vi "Test Streaming.vi"() -> ()   [LabVIEW 2021]
uses:
  <vilib>/CIF Foundation/CIF CAN RW Core/typedef/CAN Port Configuration.ctl
  <vilib>/CIF Foundation/CIF CAN RW Core/typedef/CAN Mode.ctl
  <vilib>/CIF Foundation/CIF CAN RW Core/typedef/FD Config.ctl
  <vilib>/xnet/xnet.llb/XNET Frame CAN.ctl
  <vilib>/xnet/xnet.llb/XNET Frame Type CAN.ctl
  <vilib>/CIF Foundation/CIF CAN RW Core/typedef/Statistics.ctl
  XNET CAN RW.lvclass
  C:/Program Files/National Instruments/LabVIEW 2021/vi.lib/CIF Foundation/CIF CAN RW Core/CAN_RW_CORE.lvclass
  <vilib>/CIF Foundation/CIF CAN RW Core/CAN_RW_CORE.lvclass/CAN_RW_CORE.ctl
  <vilib>/CIF Foundation/CIF CAN RW Core/Accessors/Write One Shot TX.vi
  <vilib>/CIF Foundation/CIF CAN RW Core/CAN_RW_CORE.lvclass
  D:/dev/Packages/CAN_RW_XNET/src/XNET CAN RW.lvclass
  <vilib>/CIF Foundation/CIF CAN RW Core/typedef/Communication State.ctl
  <vilib>/CIF Foundation/CIF CAN RW Core/typedef/Last Error.ctl
  <vilib>/CIF Foundation/CIF CAN RW Core/typedef/CAN Status.ctl
panel:
  out "TX CAN Status":T1
  out "RX CAN Status":T1
  out "RX Statistcs":T4
  out "TX Statistcs":T4
  in  "One Shot":bool
  in  "stop":bool
  out "RX CAN":T5[](array[typedef]) {"payload" format="%x"; "timestamp" format="%<%.7X\n%x>T"; "type" items=["CAN Data"=0, "CAN Remote"=1, "CAN Bus Error"=2, "CAN 2.0 Data"=8, "CAN FD Data"=16, "CAN FD+BRS Data"=24, "J1939 Data"=192, "Delay"=224, "Log Trigger"=225, "Start Trigger"=226]; "identifier" format="%x"}
  in  "XNET CAN Data":T5[](array[typedef])=[{"timestamp"=timestamp(3831573600 s since 1904-01-01), "payload"=[1, 2, 3, 4, 5, 6, 7, 8], "identifier"=33, "type"=16, "extended?"=TRUE, "echo?"=FALSE}, {"timestamp"=timestamp(3831570000 s since 1904-01-01), "payload"=[10, 11, 10, 13, 11, 10, 11, 14], "identifier"=82, "type"=0, "extended?"=TRUE, "echo?"=FALSE}] {"payload" format="%x"; "timestamp" format="%<%.7X\n%x>T"; "type" items=["CAN Data"=0, "CAN Remote"=1, "CAN Bus Error"=2, "CAN 2.0 Data"=8, "CAN FD Data"=16, "CAN FD+BRS Data"=24, "J1939 Data"=192, "Delay"=224, "Log Trigger"=225, "Start Trigger"=226]; "identifier" format="%x"}
  out "error out":errorcluster
  in  "Port Configuration":T7={"Mode"=enum."CAN FD", "Baud Rate"=500000, "Temination On"=TRUE, "Subordinate"=FALSE, "Echo TX"=FALSE, "FD Config"={"FD Baud Rate"=2000000, "ISO Mode"=TRUE, "BRS Enabled"=TRUE}} {"FD Config"."FD Baud Rate" format="%.0p"; "Baud Rate" format="%.0p"}
  in  "RX Initerface":string="CAN2"
  in  "TX Interface":string="CAN1"
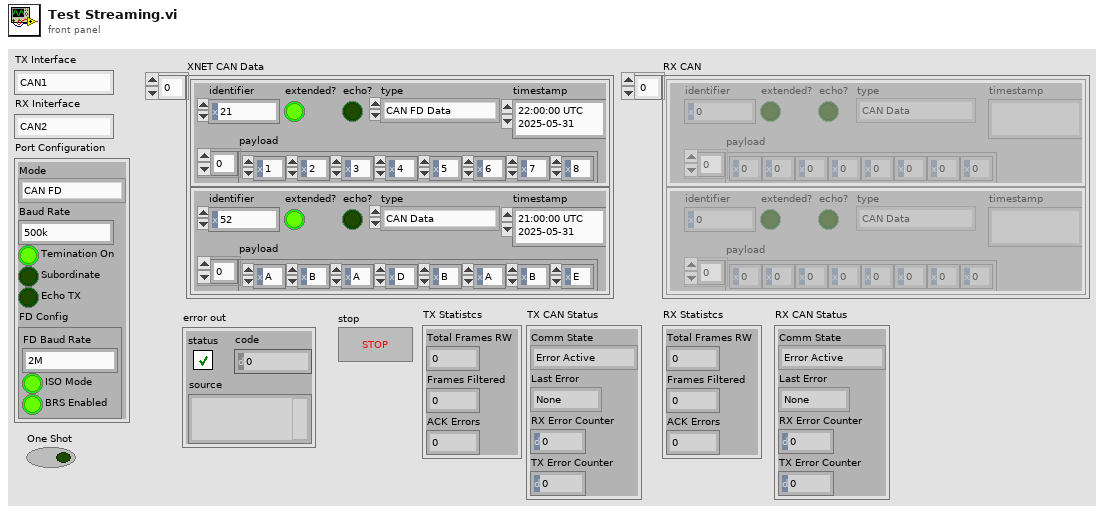
[diagram p1: front panel]
types:
  T1 = typedef "CAN_RW_CORE.lvclass/CAN Status.ctl" = cluster{"Comm State":T2, "Last Error":T3, "RX Error Counter":u8, "TX Error Counter":u8}
  T2 = typedef "CAN_RW_CORE.lvclass/Communication State.ctl" = enum16{"Error Active", "Error Passive", "Bus Off"}
  T3 = typedef "CAN_RW_CORE.lvclass/Last Error.ctl" = enum16{"None", "Stuff", "Form", "Ack", "Bit1", "Bit0", "CRC", "Unknown"}
  T4 = typedef "CAN_RW_CORE.lvclass/Statistics.ctl" = cluster{"Total Frames RW":u32, "Frames Filtered ":u32, "ACK Errors":u32}
  T5 = typedef "XNET Frame CAN.ctl" = cluster{"timestamp":timestamp, "payload":u8[], "identifier":u32, "type":T6, "extended?":bool, "echo?":bool}
  T6 = typedef "XNET Frame Type CAN.ctl" = u8
  T7 = typedef "CAN_RW_CORE.lvclass/CAN Port Configuration.ctl" = cluster{"Mode":T8, "Baud Rate":u64, "Temination On":bool, "Subordinate":bool, "Echo TX":bool, "FD Config":T9}
  T8 = typedef "CAN_RW_CORE.lvclass/CAN Mode.ctl" = enum16{"CAN 2.0", "CAN FD"}
  T9 = typedef "CAN_RW_CORE.lvclass/FD Config.ctl" = cluster{"FD Baud Rate":u64, "ISO Mode":bool, "BRS Enabled":bool}
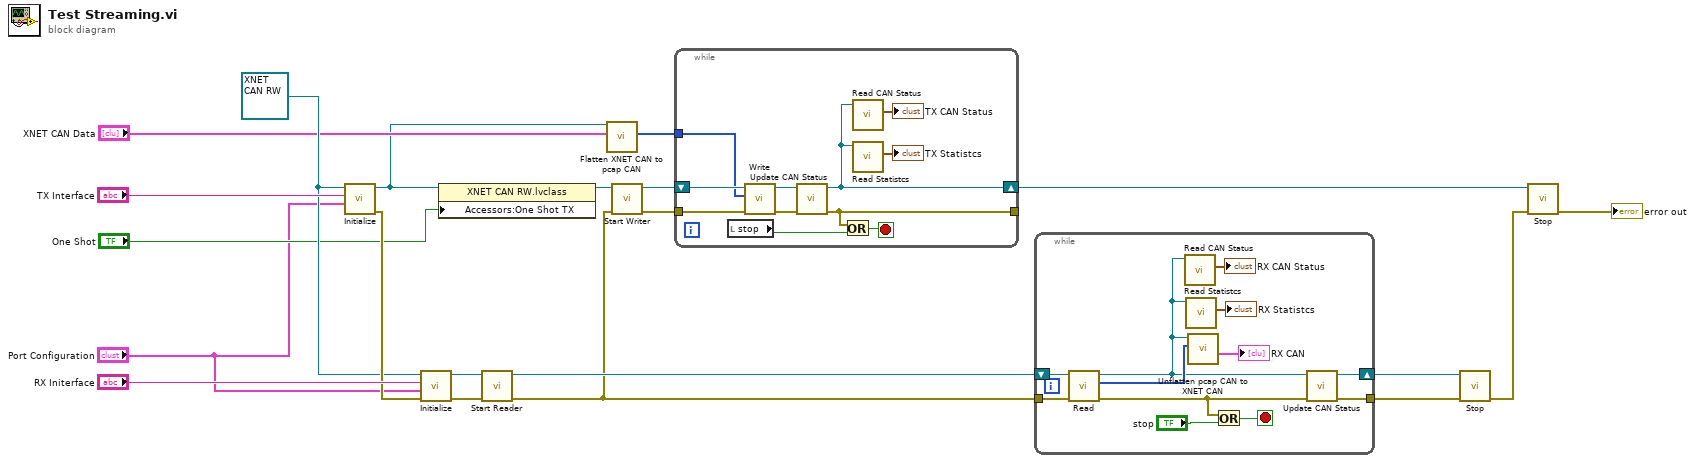
[diagram p0: block diagram]
diagram:
  w11 = refnum<class "XNET CAN RW.lvclass"> refnum ("CAN_Logic in")
  n1 = call "Initialize.vi"("Port Configuration"="Port Configuration", "Interface"="TX Interface", "XNET_CAN_RW in"=w11) -> ("error out"=w20:errorcluster, "XNET_CAN_RW out"=w4:refnum<class "XNET CAN RW.lvclass">)  [unwired: 7 in]
  n2 = call "Initialize.vi"("error in (no error)"=w20, "Port Configuration"="Port Configuration", "Interface"="RX Initerface", "XNET_CAN_RW in"=w11) -> ("error out"=w18:errorcluster, "XNET_CAN_RW out"=w19:refnum<class "XNET CAN RW.lvclass">)  [unwired: 6 in]
  n3 = property class="XNET CAN RW.lvclass"(reference=w4, "Accessors:One Shot TX"="One Shot") -> (reference out=w3:refnum<class "XNET CAN RW.lvclass">)  [unwired: 1 in, 1 out]
  n4 = call-dynamic "Start Reader.vi"("error in (no error)"=w18, "XNET_CAN_RW in"=w19) -> ("error out"=w6:errorcluster, "XNET_CAN_RW out"=w8:refnum<class "XNET CAN RW.lvclass">)  [unwired: 8 in]
  n5 = call "Flatten XNET CAN to pcap CAN.vi"("XNET CAN Data"="XNET CAN Data", "XNET_CAN_RW in"=w4) -> ("pcap CAN DATA"=w9:u8[])  [unwired: 7 in, 2 out]
  n6 = call-dynamic "Start Writer.vi"("error in (no error)"=w6, "XNET_CAN_RW in"=w3) -> ("error out"=w16:errorcluster, "XNET_CAN_RW out"=w17:refnum<class "XNET CAN RW.lvclass">)  [unwired: 8 in]
  n7 = while {
    tunnel: w9 -> [w30]
    shift-right: [w23] -> w13
    shift-left: w17 -> [w32]
    tunnel: w16 -> [w31]
    tunnel: [w24] -> _
    stop <- w29 stop-if-true
    n8 = local read "stop"() -> (w27:bool)
    n9 = call-dynamic "Write.vi"("error in (no error)"=w31, "pcap CAN DATA in"=w30, "XNET_CAN_RW in"=w32) -> ("error out"=w25:errorcluster, "XNET_CAN_RW out"=w26:refnum<class "XNET CAN RW.lvclass">)  [unwired: 6 in, 1 out]
    n10 = call "Update CAN Status.vi"("error in (no error)"=w25, "XNET CAN RW in"=w26) -> ("error out"=w24:errorcluster, "XNET CAN RW out"=w23:refnum<class "XNET CAN RW.lvclass">)  [unwired: 8 in]
    n11 = Or(x=w24, y=w27) -> (x .or. y?=w29:bool)
    n12 = call <vilib>:"Read CAN Status.vi"("CAN_RW_CORE in"=w23) -> ("CAN Status"=→"TX CAN Status":T1)  [unwired: 8 in, 2 out]
    n13 = call <vilib>:"Read Statistcs.vi"("CAN_RW_CORE in"=w23) -> ("Statistcs"=→"TX Statistcs":T4)  [unwired: 8 in, 2 out]
  }
  n14 = while {
    shift-right: [w37] -> w15
    shift-left: w8 -> [w43]
    tunnel: w6 -> [w42]
    tunnel: [w36] -> w14
    stop <- w40 stop-if-true
    n15 = call-dynamic "Read.vi"("error in (no error)"=w42, "XNET_CAN_RW in"=w43) -> ("error out"=w35:errorcluster, "pcap CAN Data"=w41:u8[], "XNET_CAN_RW out"=w34:refnum<class "XNET CAN RW.lvclass">)  [unwired: 5 in, 2 out]
    n16 = call <vilib>:"Read CAN Status.vi"("CAN_RW_CORE in"=w34) -> ("CAN Status"=→"RX CAN Status":T1)  [unwired: 8 in, 2 out]
    n17 = call <vilib>:"Read Statistcs.vi"("CAN_RW_CORE in"=w34) -> ("Statistcs"=→"RX Statistcs":T4)  [unwired: 8 in, 2 out]
    n18 = call "Unflatten pcap CAN to XNET CAN.vi"("pcap CAN DATA in"=w41, "XNET_CAN_RW in"=w34) -> ("XNET CAN Data"=→"RX CAN":T5[])  [unwired: 4 in, 5 out]
    n19 = Or(x=w35, y="stop") -> (x .or. y?=w40:bool)
    n20 = call "Update CAN Status.vi"("error in (no error)"=w35, "XNET CAN RW in"=w34) -> ("error out"=w36:errorcluster, "XNET CAN RW out"=w37:refnum<class "XNET CAN RW.lvclass">)  [unwired: 8 in]
  }
  n21 = call-dynamic "Stop.vi"("error in (no error)"=w14, "XNET_CAN_RW in"=w15) -> ("error out"=w7:errorcluster)  [unwired: 8 in, 1 out]
  n22 = call-dynamic "Stop.vi"("error in (no error)"=w7, "XNET_CAN_RW in"=w13) -> ("error out"=→"error out":errorcluster)  [unwired: 8 in, 1 out]
